vi "Scan Sample.vi"(0 "Czas naœwietlania (us)":dbl, 5 "pixels x":i32=128, 7 "pixels y":i32=128, 9 "Zakres skanowania min":dbl, 11 "Zakres skanowania max":dbl, 12 "error in":errorcluster) -> (4 "data":dbl[](array[numeric]) format="%0.2f", 15 "error out":errorcluster)   [LabVIEW 2021]
uses:
  <vilib>/DAQmx/read.llb/DAQmx Read (Analog 1D DBL 1Chan NSamp).vi
  <vilib>/Analysis/1siggen.llb/Ramp Pattern by Samples.vi
  <vilib>/DAQmx/write.llb/DAQmx Write (Analog 2D DBL NChan NSamp).vi
  <vilib>/DAQmx/create/channels.llb/DAQmx Create Channel (AO-Voltage-Basic).vi
  <vilib>/DAQmx/configure/timing.llb/DAQmx Timing (Sample Clock).vi
  <vilib>/DAQmx/create/channels.llb/DAQmx Create Channel (AI-Voltage-Basic).vi
  <vilib>/DAQmx/miscellaneous.llb/DAQmx Fill In Error Info.vi
  <vilib>/measure/NI_MABase.lvlib
  <vilib>/Analysis/NI_AALBase.lvlib
  <resource>/objmgr/daqmx.rc
panel:
  out "Intensity Graph":dbl[][](graph)
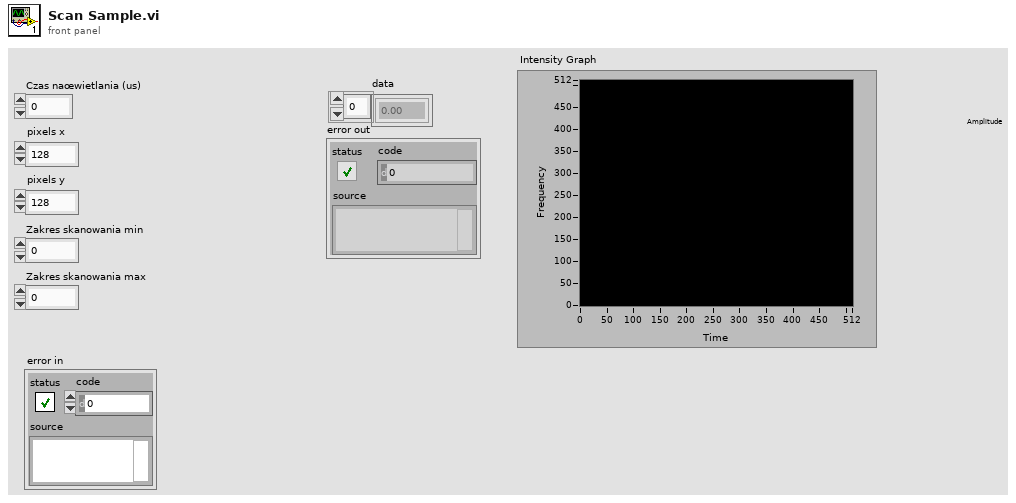
[diagram p1: front panel]
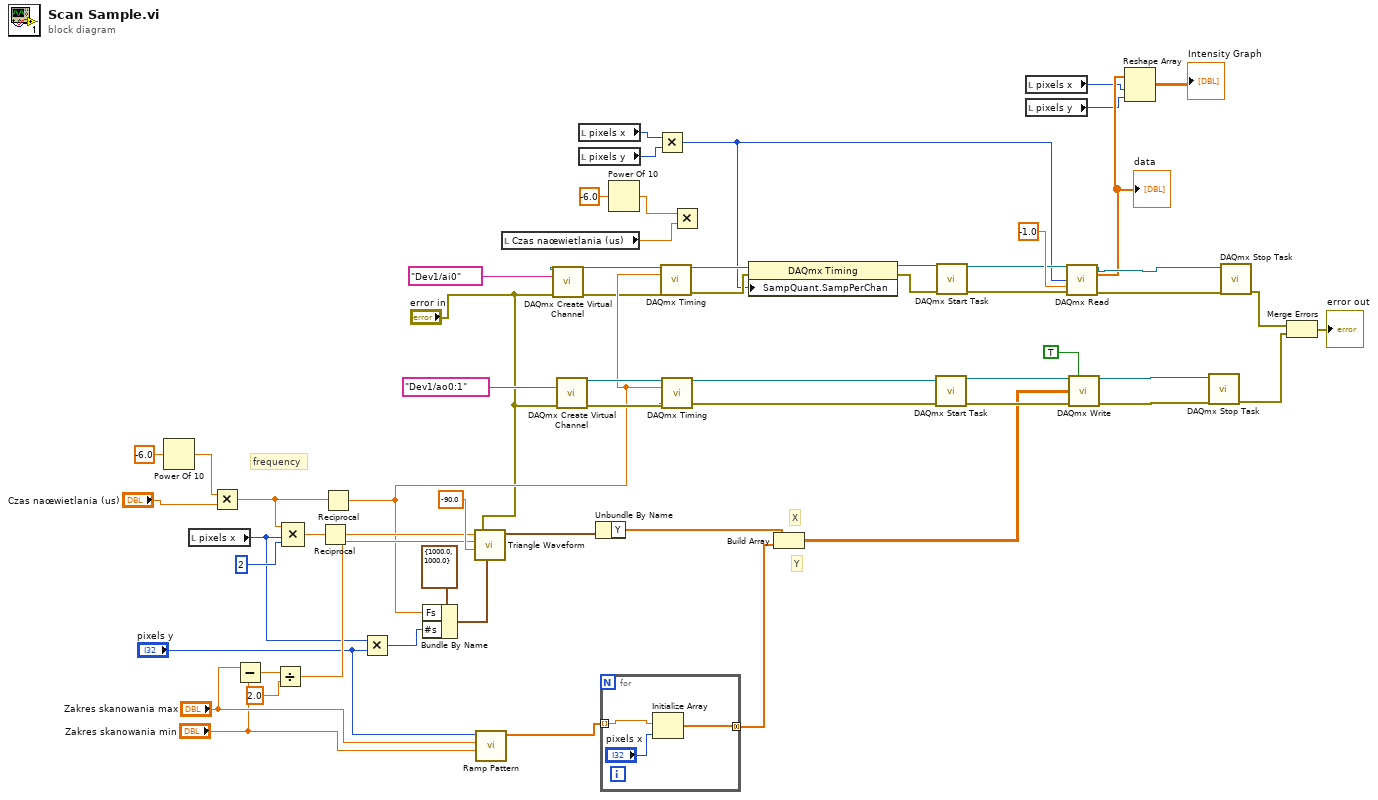
[diagram p0: block diagram]
diagram:
  # "Y"
  # "X"
  # "frequency"
  n1 = Power Of 10(x=-6.0) -> (10^x=w31:dbl)
  n2 = local read "pixels x"() -> (w45:i32)
  n3 = Multiply(x=w31, y="Czas naœwietlania (us)") -> (x*y=w30:dbl)
  n4 = Subtract(x="Zakres skanowania max", y="Zakres skanowania min") -> (x-y=w50:dbl)
  n5 = Divide(x=w50, y=2.0) -> (x/y=w48:dbl)
  n6 = Compound Arithmetic op=MULTIPLY(w30, w45, 2) -> (w54:dbl)
  n7 = Reciprocal(x=w54) -> (1/x=w53:dbl)
  n8 = Reciprocal(x=w30) -> (1/x=w28:dbl)
  n9 = Multiply(x=w45, y="pixels y") -> (x*y=w44:i32)
  n10 = Bundle By Name(cluster=cluster{"Fs":dbl, "#s":dbl} {"Fs"=1000.0, "#s"=1000.0} ("sampling info"), "Fs"=w28, "#s"=w44) -> (w43:cluster{"Fs":dbl, "#s":dbl})
  n11 = call <vilib>:"Triangle Waveform.vi"("sampling info"=w43, "error in (no error)"="error in", "phase"=-90.0, "amplitude"=w48, "frequency"=w53) -> ("signal out"=w59:waveform(dbl))  [unwired: 5 in, 1 out]
  n12 = call-poly <vilib>:"Ramp Pattern.vi"("start"="Zakres skanowania min", "end"="Zakres skanowania max", "samples"="pixels y") -> ("Ramp Pattern"=w60:dbl[])  [unwired: 7 in, 1 out]
  n13 = local read "Czas naœwietlania (us)"() -> (w21:dbl)
  n14 = call-poly <vilib>:"DAQmx Create Virtual Channel.vi"("physical channels"=tag "Dev1/ai0", "error in"="error in") -> ("task out"=w27:refnum<k21>, "error out"=w26:errorcluster)  [unwired: 12 in]
  n15 = call-poly <vilib>:"DAQmx Create Virtual Channel.vi"("physical channels"=tag "Dev1/ao0:1", "error in"="error in") -> ("task out"=w41:refnum<k21>, "error out"=w42:errorcluster)  [unwired: 12 in]
  n16 = local read "pixels x"() -> (w25:i32)
  n17 = local read "pixels y"() -> (w24:i32)
  n18 = Unbundle By Name(w59) -> ("Y"=w58:dbl[])
  n19 = for {
    tunnel: w60 -> [w63] mode=indexing
    tunnel: [w62] -> w57 mode=concatenating
    n20 = Initialize Array(w63, "pixels x") -> (w62:dbl[])
  }
  n21 = Power Of 10(x=-6.0) -> (10^x=w22:dbl)
  n22 = Multiply(x=w25, y=w24) -> (x*y=w4:i32)
  n23 = call-poly <vilib>:"DAQmx Timing.vi"("task/channels in"=w27, "rate"=w28, "error in"=w26) -> ("task out"=w6:refnum<k21>, "error out"=w5:errorcluster)  [unwired: 11 in]
  n24 = call-poly <vilib>:"DAQmx Timing.vi"("task/channels in"=w41, "rate"=w28, "error in"=w42) -> ("task out"=w39:refnum<k21>, "error out"=w38:errorcluster)  [unwired: 11 in]
  n25 = Multiply(x=w22, y=w21) -> ()  [unwired: 1 out]
  n26 = property class="DAQmx Timing"(reference=w6, error in=w5, "SampQuant.SampPerChan"=w4) -> (reference out=w3:refnum<k21>, error out=w2:errorcluster)
  n27 = Build Array(w58, w57) -> (w35:dbl[][])
  n28 = call <vilib>:"DAQmx Start Task.vi"("task/channels in"=w39, "error in"=w38) -> ("task out"=w36:refnum<k21>, "error out"=w37:errorcluster)  [unwired: 12 in]
  n29 = call <vilib>:"DAQmx Start Task.vi"("task/channels in"=w3, "error in"=w2) -> ("task out"=w7:refnum<k21>, "error out"=w8:errorcluster)  [unwired: 12 in]
  n30 = local read "pixels x"() -> (w14:i32)
  n31 = local read "pixels y"() -> (w13:i32)
  n32 = call-poly <vilib>:"DAQmx Read.vi"("task/channels in"=w7, "number of samples per channel"=w4, "timeout"=-1.0, "error in"=w8) -> ("task out"=w16:refnum<k21>, "data"=w15:dbl[], "error out"=w17:errorcluster)  [unwired: 9 in]
  "data" <- w15
  n33 = call-poly <vilib>:"DAQmx Write.vi"("task/channels in"=w36, "auto start"=TRUE, "data"=w35, "error in"=w37) -> ("task out"=w18:refnum<k21>, "error out"=w19:errorcluster)  [unwired: 9 in, 1 out]
  n34 = Reshape Array(w15, w14, w13) -> (→"Intensity Graph":dbl[][])
  n35 = call <vilib>:"DAQmx Stop Task.vi"("task/channels in"=w18, "error in"=w19) -> ("error out"=w10:errorcluster)  [unwired: 12 in, 1 out]
  n36 = call <vilib>:"DAQmx Stop Task.vi"("task/channels in"=w16, "error in"=w17) -> ("error out"=w11:errorcluster)  [unwired: 12 in, 1 out]
  n37 = Merge Errors(w11, w10) -> (→"error out":errorcluster)
